vi "Upload_test_VI _20230224.vi"(8 "error in":errorcluster, 11 "SHz_selection":enum16{"10k", "100k"}(ring)) -> (0 "error out":errorcluster, 2 "selected F_array_Link":path[](array[path]), 3 "selected folder_List":string[](array[string]))   [LabVIEW 2018]
panel:
  out "present_s_path":path
  out "S_path":path[](array[path])
  in  "Server selection":u16(ring) items=["Rackstation", "QTserver", "QDserver", "D:\\", "C:\\", "SQserver"]
  in  "Add All Sample":bool
  in  "Add All":bool
  out "FOL#":i32
  out "x-1":u32
  out "SIDE":i32
  in  "Scrollbar V":i32(c297)
  out "Selected EX#":i32
  out "element":string
  in  "END":bool
  in  "All_Clear":bool
  in  "EX_IDX":i32
  out "Height":u32
  out "Top":i32
  out "Vertical":i32
  in  "selection":u16(ring) items=["backup (Rackstation)", "BR", "cadet", "COVID19", "Gynecologic Cancer", "HU", "KATO", "KATO2", "KATO3", "komoto", "Konno", "Kumamoto", "Kumamoto_N", "Lee", "Lee2", "Lee3", "LG_EX", "Lipid", "Numata_CHR", "Numata_MF", "Numata_N", "oligopeptide", "Pan_Cancer_N2", "Phi174", "Ryu", "Smoking"]
  out "1folder names":string[](array[string])
  out "Folder_List":string[](array[string])
  out "F_array_Link":path[](array[path])
  out "2folder_name":string[](array[string])
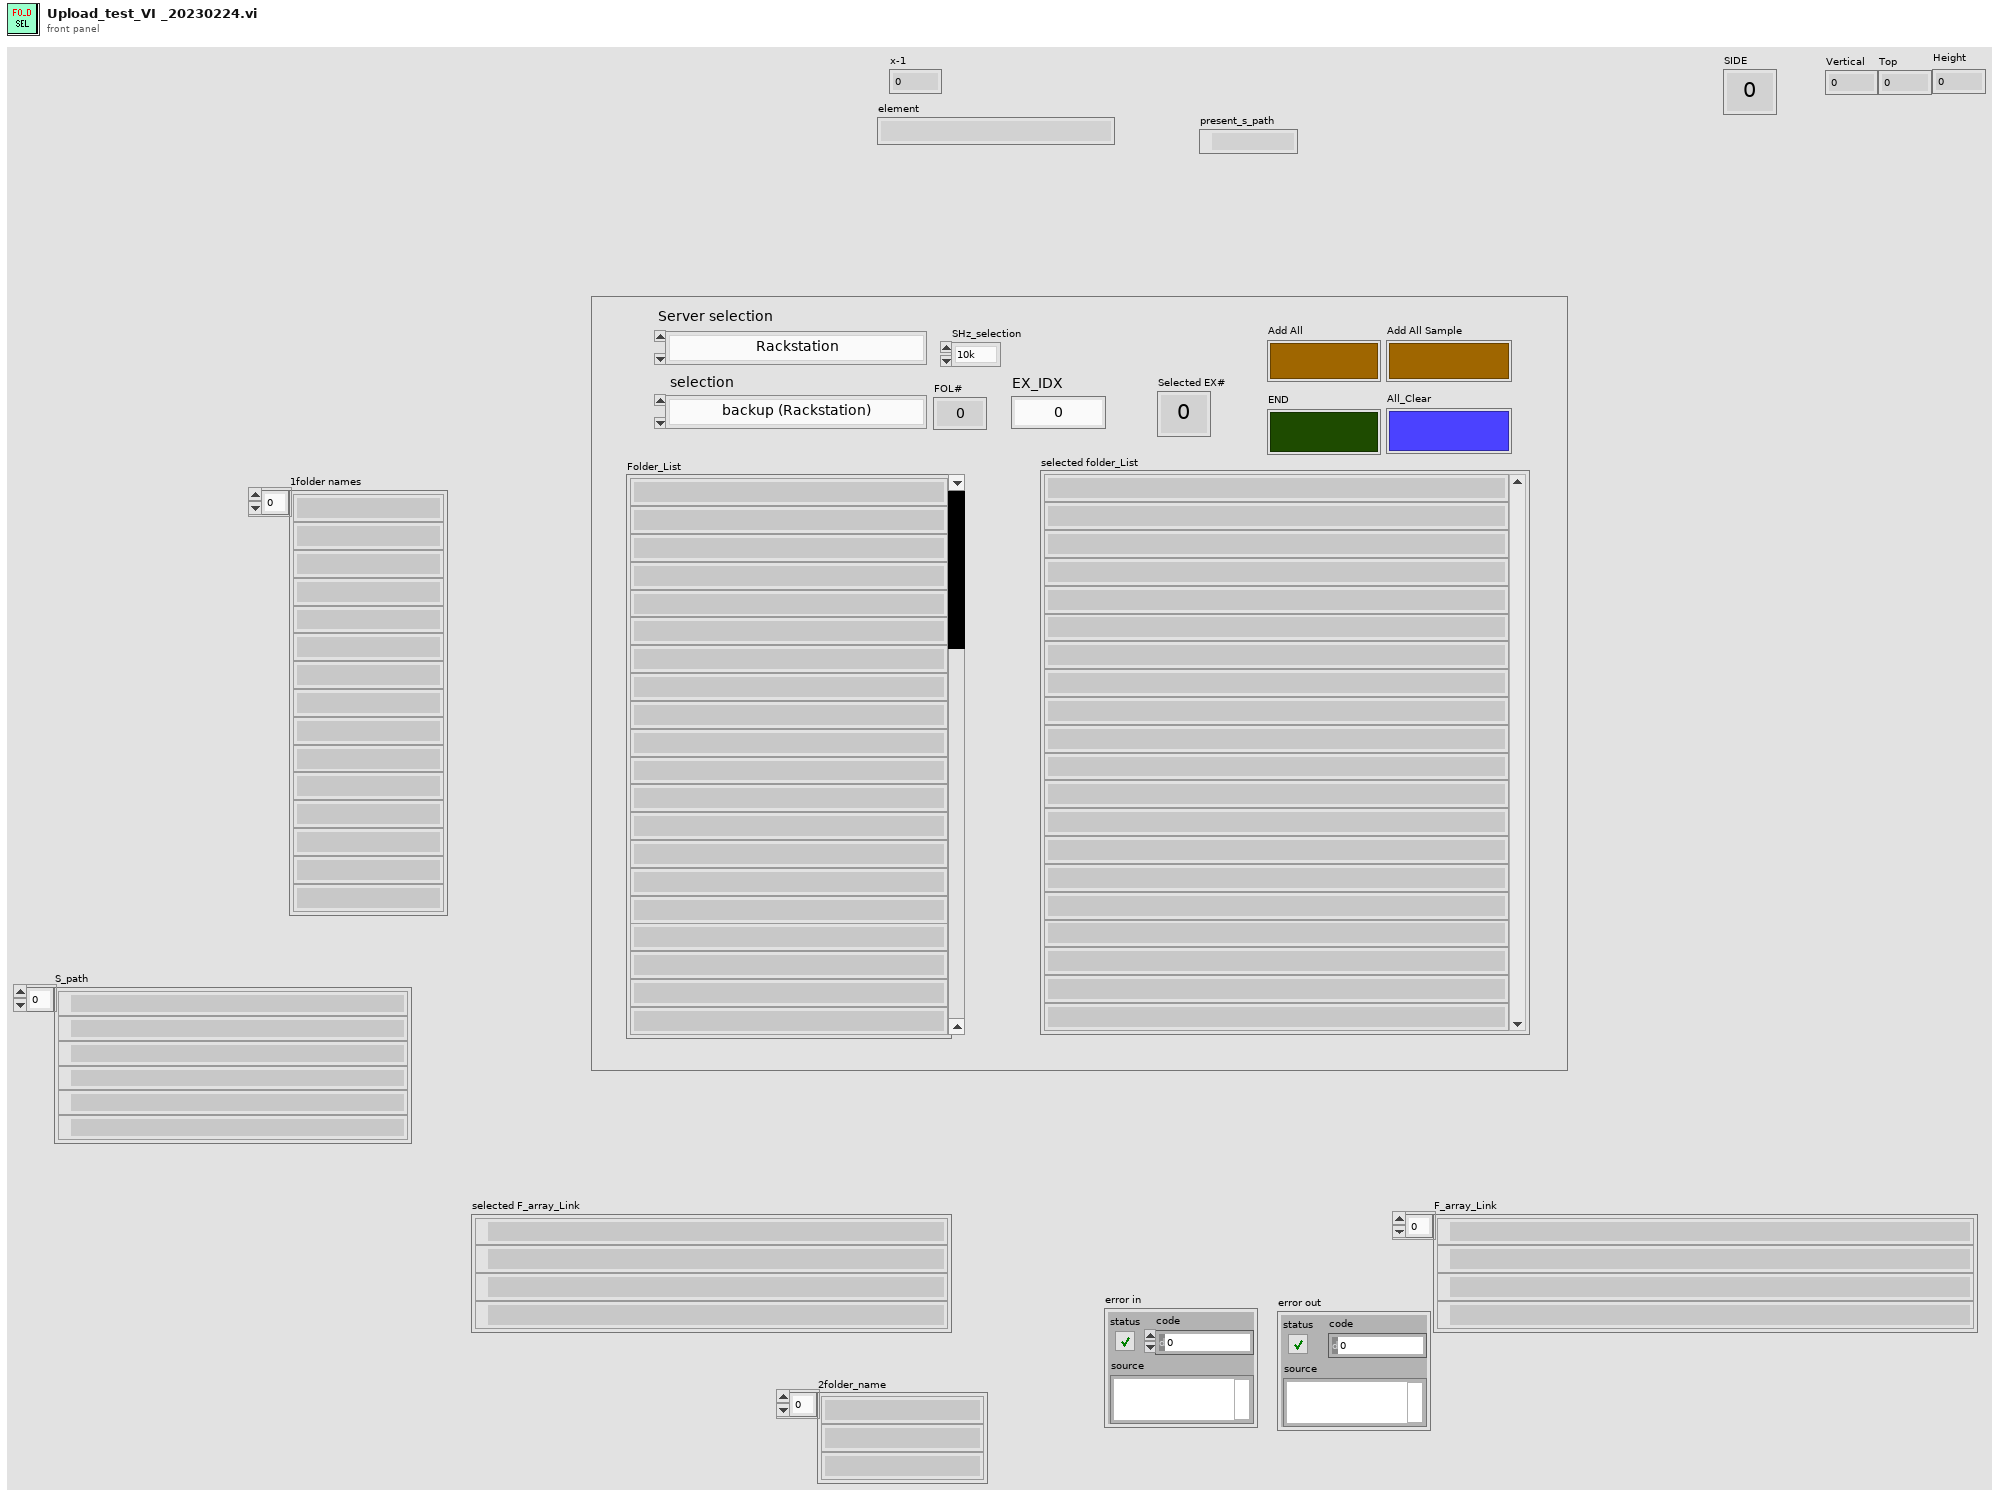
[diagram p1: front panel]
types:
  T1 = typedef "LVPoint32TypeDef.ctl" = cluster{"Horizontal":i32, "Vertical":i32}
  T2 = typedef "LVPositionTypeDef.ctl" = cluster{"Left":i32, "Top":i32}
  T3 = typedef "LVBoundsTypeDef.ctl" = cluster{"Width":u32, "Height":u32}
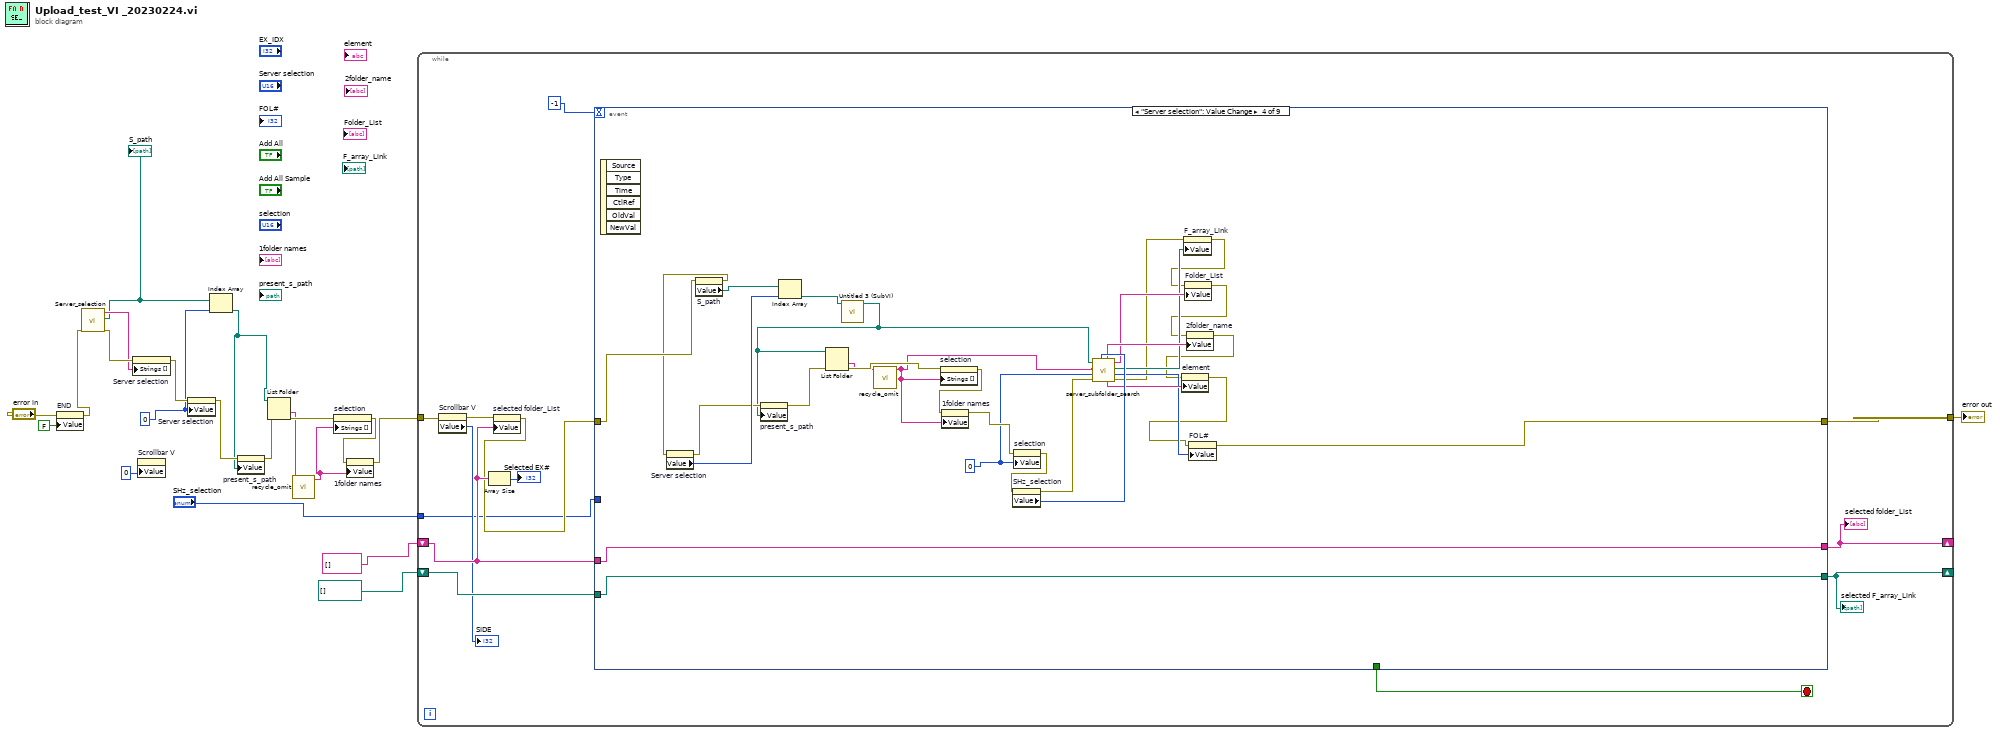
[diagram p0: block diagram]
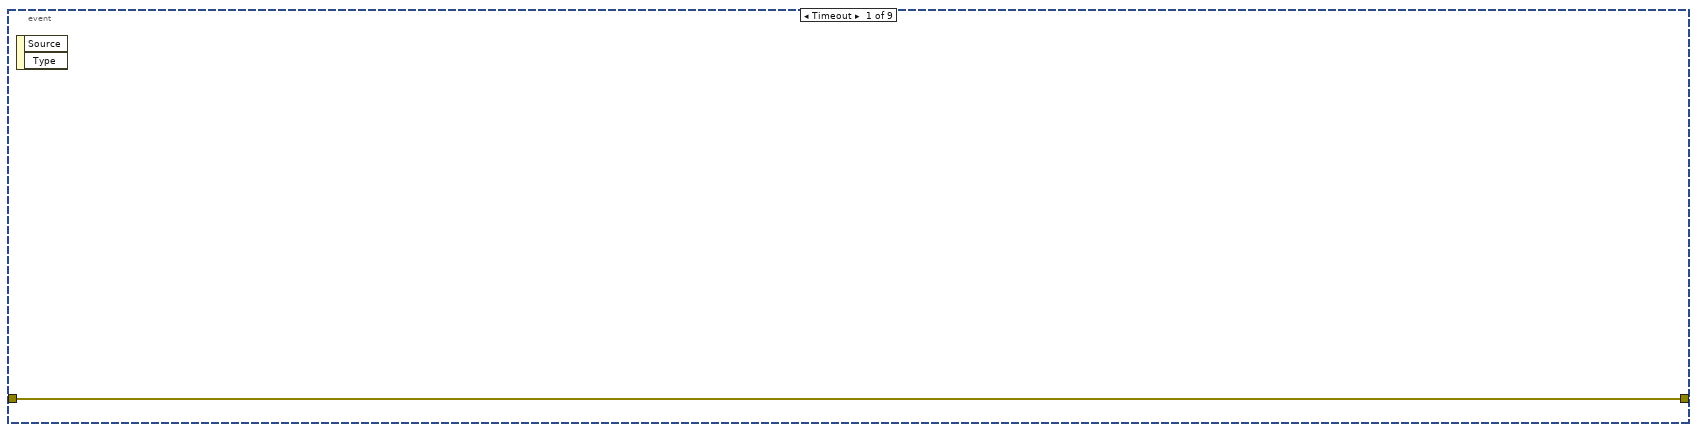
[diagram p2: hidden frame]
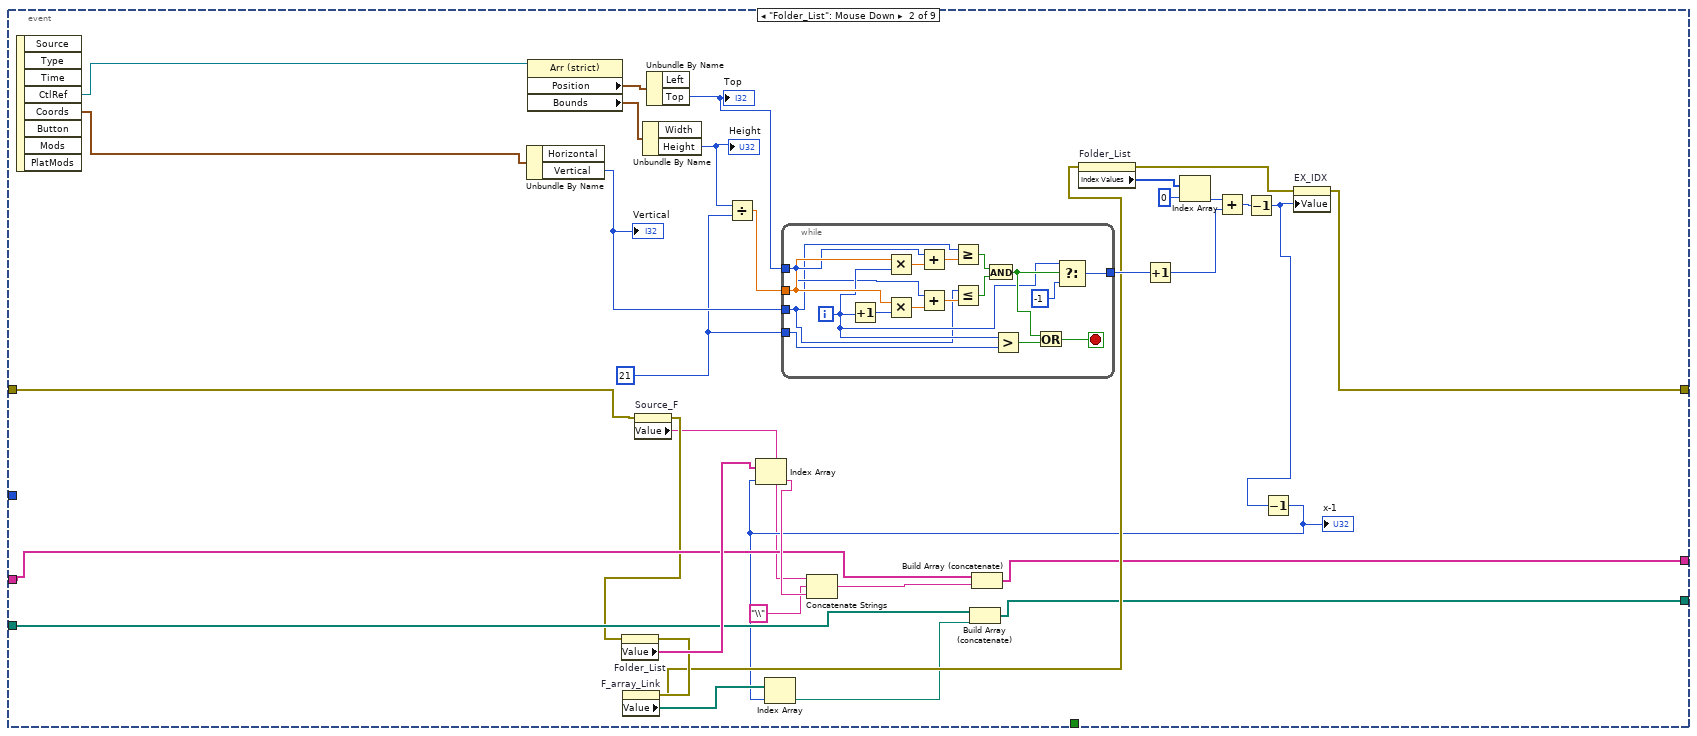
[diagram p3: hidden frame]
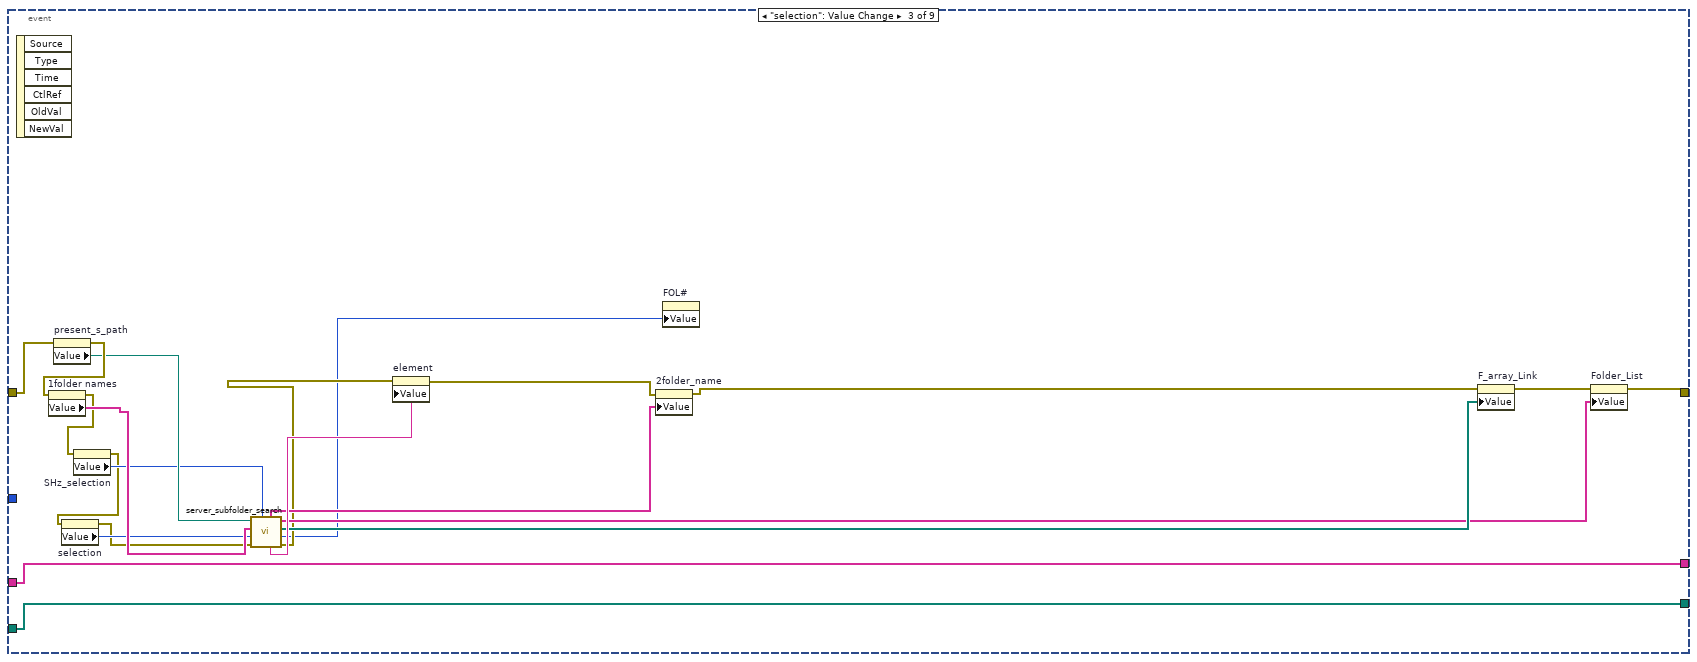
[diagram p4: hidden frame]
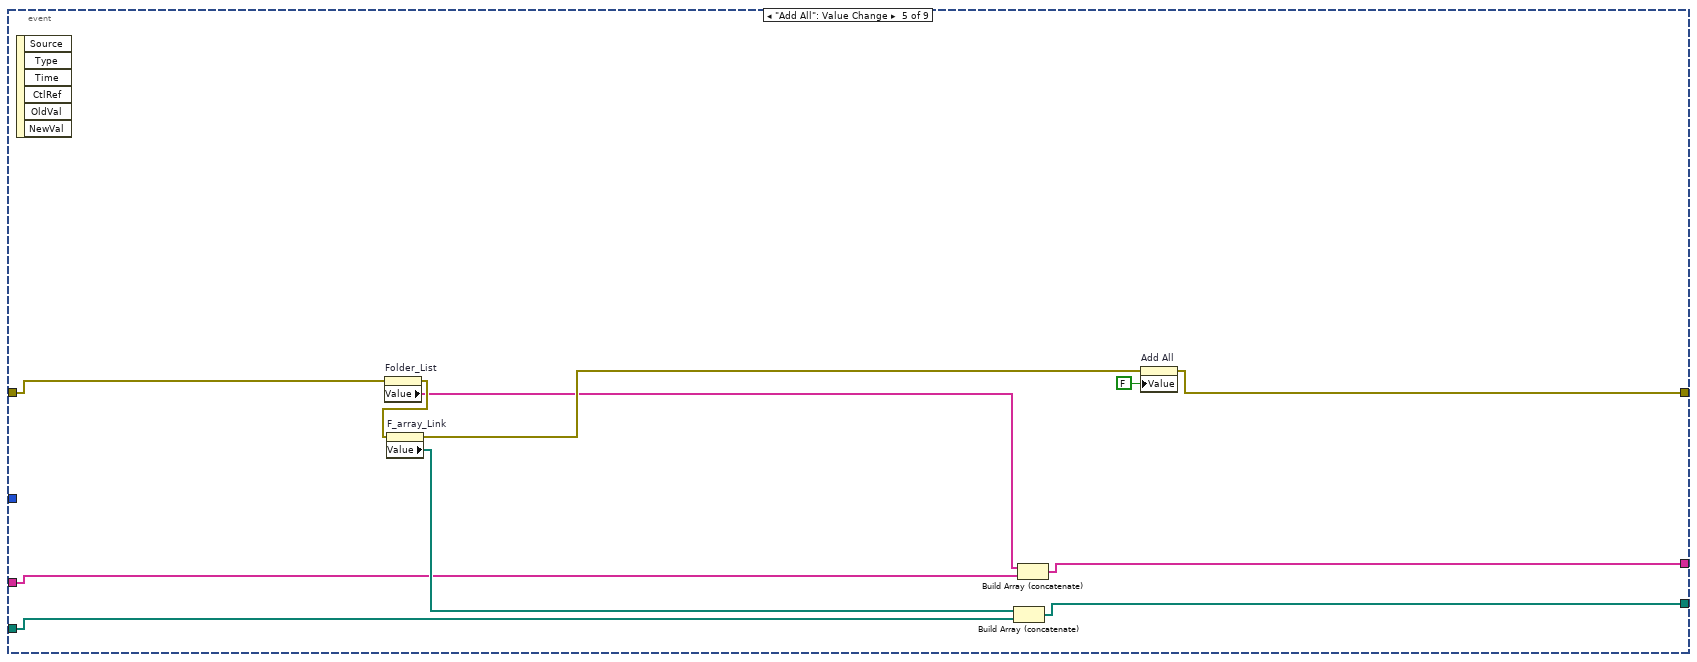
[diagram p5: hidden frame]
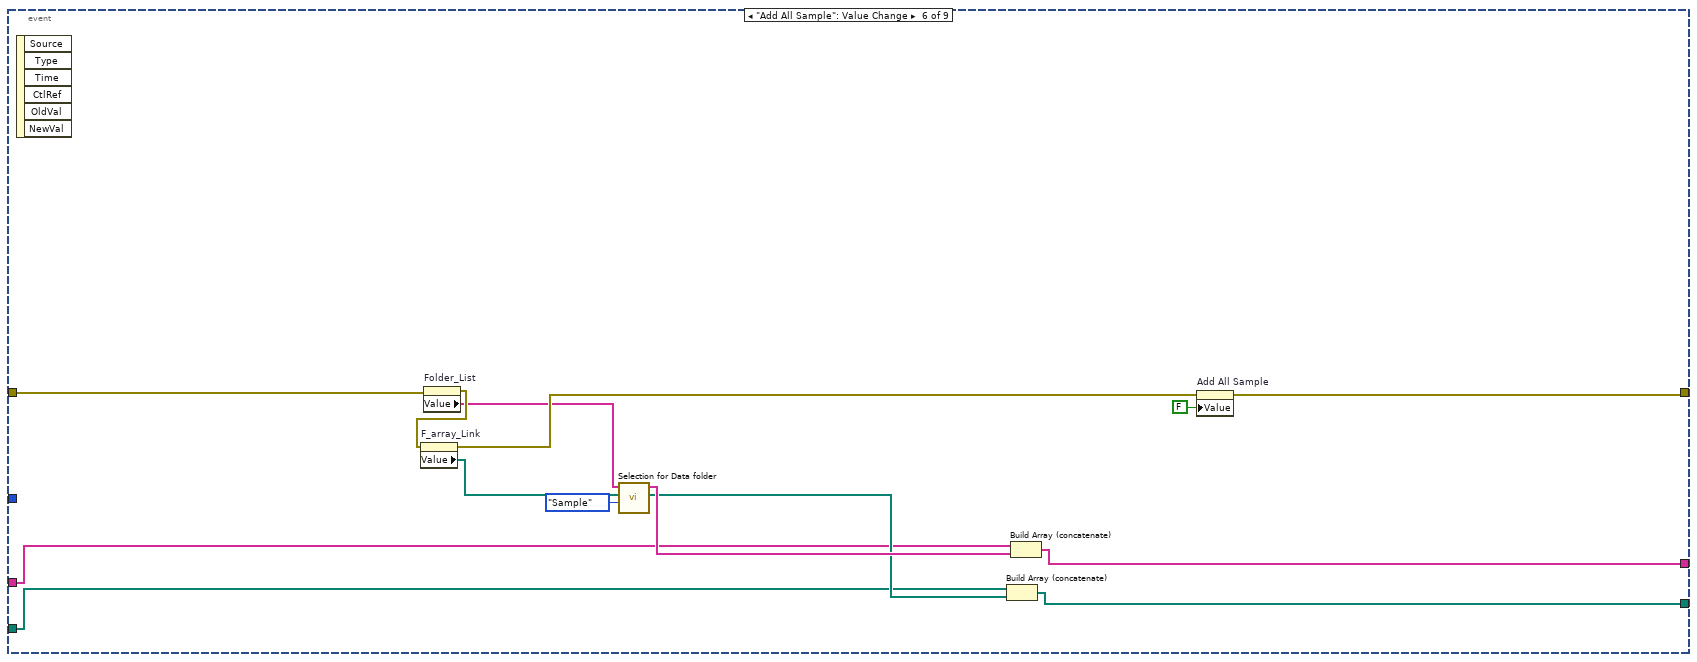
[diagram p6: hidden frame]
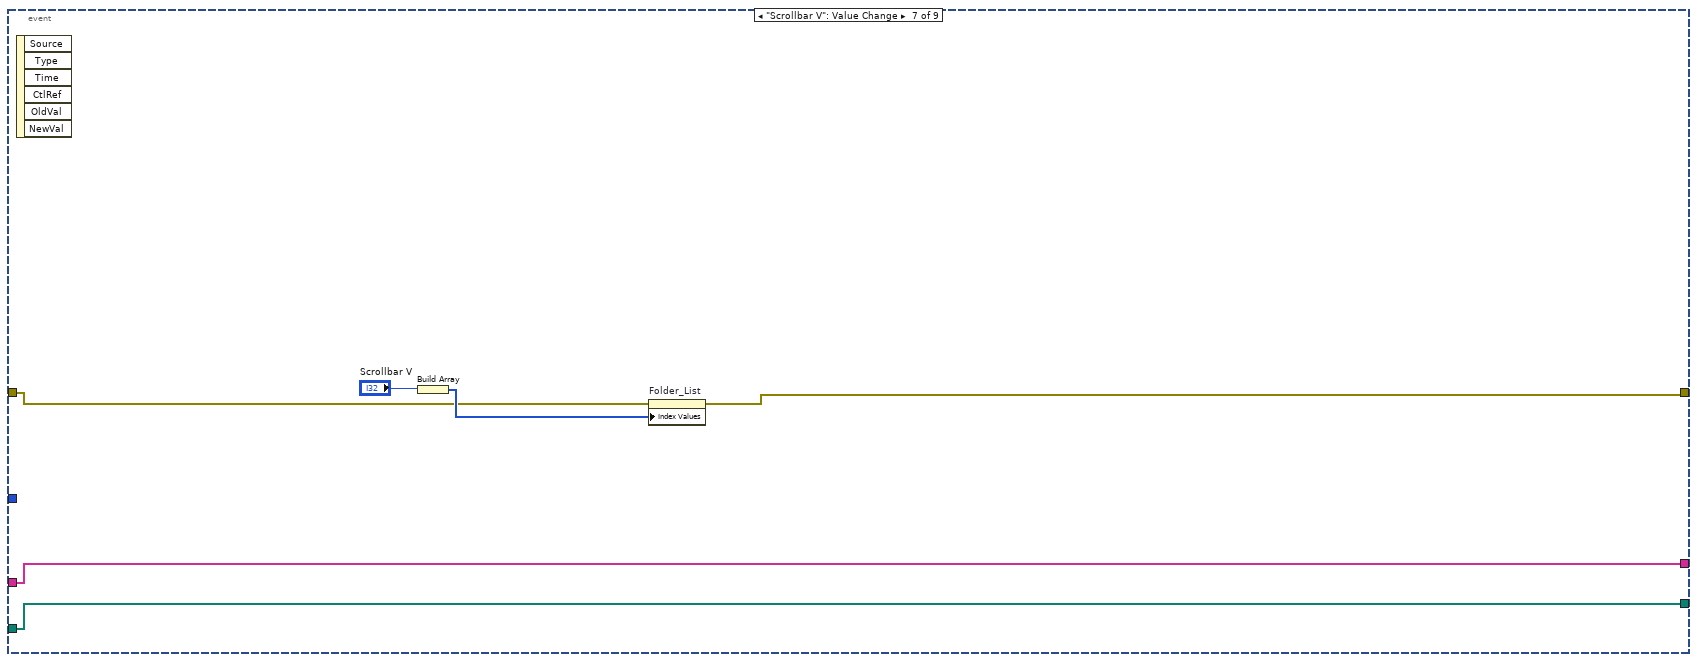
[diagram p7: hidden frame]
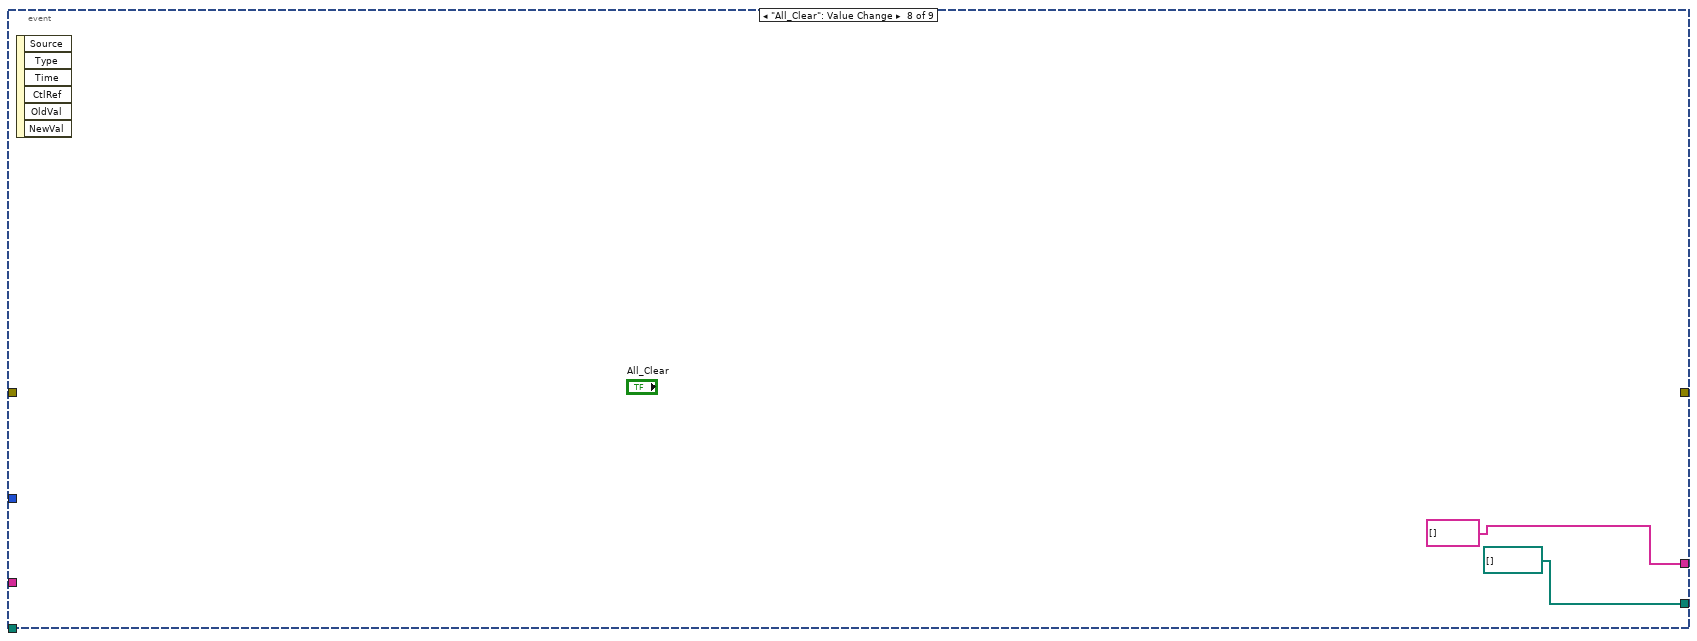
[diagram p8: hidden frame]
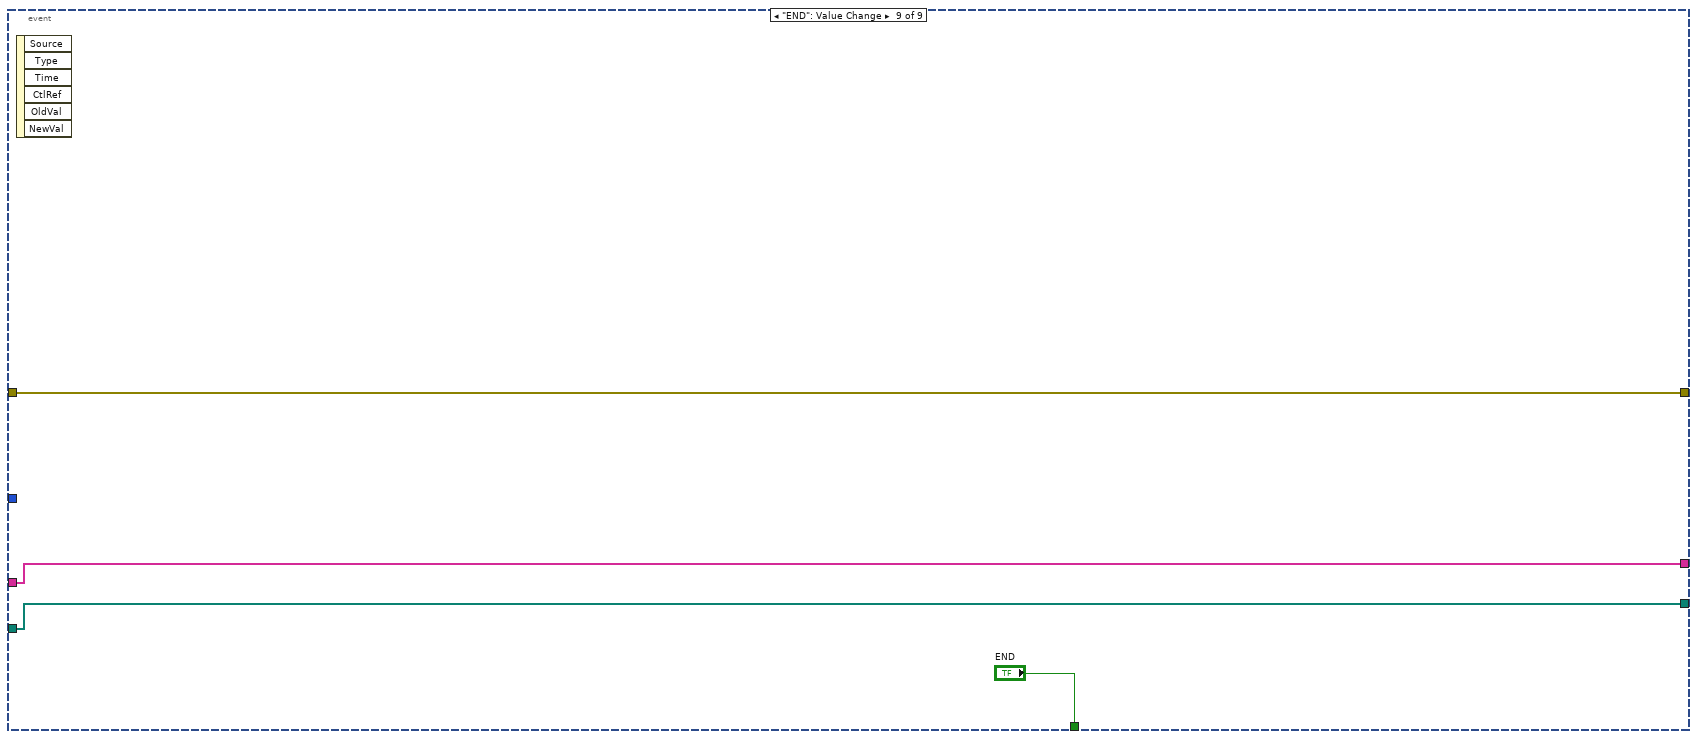
[diagram p9: hidden frame]
diagram:
  w7 = 0
  n1 = property on="END" class="Bool (strict)"(error in="error in", "Value"=FALSE ("END")) -> (error out=w12:errorcluster)  [unwired: 1 in, 1 out]
  n2 = call "Server_selection.vi"("error in (no error)"=w12) -> ("error out"=w11:errorcluster, "path 2"=w8:path[], "server_name_list"=w10:string[])  [unwired: 8 in]
  "S_path" <- w8
  n3 = property on="Server selection" class="Ring (strict)"(error in=w11, "Strings []"=w10) -> (error out=w9:errorcluster)  [unwired: 1 in, 1 out]
  n4 = property on="Scrollbar V" class="Scroll (strict)"("Value"=0 ("Scrollbar V")) -> ()  [unwired: 2 in, 2 out]
  n5 = property on="Server selection" class="Ring (strict)"(error in=w9, "Value"=w7) -> (error out=w3:errorcluster)  [unwired: 1 in, 1 out]
  n6 = Index Array(array=w8, index=w7) -> (element=w1:path)
  n7 = property on="present_s_path" class="Path"(error in=w3, "Value"=w1) -> (error out=w2:errorcluster)  [unwired: 1 in, 1 out]
  n8 = List Folder(path=w1, error in=w2) -> (folder names=w16:string[], error out=w21:errorcluster)  [unwired: 2 in, 2 out]
  n9 = call "recycle_omit.vi"("1folder names"=w16) -> ("Array"=w6:string[])  [unwired: 10 in]
  n10 = property on="selection" class="Ring (strict)"(error in=w21, "Strings []"=w6) -> (error out=w5:errorcluster)  [unwired: 1 in, 1 out]
  n11 = property on="1folder names" class="Arr (strict)"(error in=w5, "Value"=w6) -> (error out=w4:errorcluster)  [unwired: 1 in, 1 out]
  n12 = while {
    tunnel: w4 -> [w27]
    tunnel: [w34] -> w20
    shift-right: [w24] -> _
    shift-left: string[] [] -> [w29]
    shift-right: [w30] -> _
    shift-left: path[] [] -> [w31]
    tunnel: "SHz_selection" -> [w22]
    stop <- w32 stop-if-true
    n13 = property on="Scrollbar V" class="Scroll (strict)"(error in=w27) -> (error out=w26:errorcluster, "Value"=→"SIDE":i32)  [unwired: 1 in, 1 out]
    n14 = Array Size(array=w29) -> (size(s)=→"Selected EX#":i32)
    n15 = property on="selected folder_List" class="Arr (strict)"(error in=w26, "Value"=w29) -> (error out=w23:errorcluster)  [unwired: 1 in, 1 out]
    n16 = event shown="[3] \"Server selection\": Value Change" {
      selector: _ -> [_ _ _ _ _ _ _ _ _]
      dyn-events: _ -> [_ _ _ _ _ _ _ _ _]
      timeout: -1 -> [_ _ _ _ _ _ _ _ _]
      tunnel: w23 -> [w35 w39 w104 w135 w148 w161 w167 _ w171]
      tunnel: [w35 w41 w107 w108 w144 w158 w166 _ w171] -> w34
      tunnel: w29 -> [_ w44 w106 w136 w138 w149 w164 _ w173]
      tunnel: [_ w43 w106 w136 w142 w152 w164 string[] [] w173] -> w24
      tunnel: [_ _ _ _ _ _ _ _ "END"] -> w32
      tunnel: w31 -> [_ w45 w105 w137 w139 w150 w163 _ w172]
      tunnel: [_ w42 w105 w137 w141 w151 w163 path[] [] w172] -> w30
      tunnel: w22 -> [_ _ _ _ _ _ _ _ _]
      event Timeout {
        n17 = event-data() -> ()  [unwired: 1 in, 2 out]
      }
      event "Folder_List": Mouse Down {
        w49 = 21 ("f")
        n18 = event-data() -> ("CtlRef"=w46:refnum<vi>, "Coords"=w47:T1)  [unwired: 1 in, 6 out]
        n19 = Unbundle By Name(w47) -> ("Vertical"=w66:i32)  [unwired: 1 out]
        "Vertical" <- w66
        n20 = property class="Arr (strict)"(reference=w46) -> ("Position"=w68:T2, "Bounds"=w67:T3)  [unwired: 1 in, 2 out]
        n21 = property on="Source_F" class="Str"(error in=w39) -> (error out=w38:errorcluster, "Value"=w37:string)  [unwired: 1 in, 1 out]
        n22 = property on="Folder_List" class="Arr (strict)"(error in=w38) -> (error out=w54:errorcluster, "Value"=w58:string[])  [unwired: 1 in, 1 out]
        n23 = property on="F_array_Link" class="Arr (strict)"(error in=w54) -> (error out=w53:errorcluster, "Value"=w52:path[])  [unwired: 1 in, 1 out]
        n24 = Unbundle By Name(w67) -> ("Height"=w65:u32)  [unwired: 1 out]
        "Height" <- w65
        n25 = Unbundle By Name(w68) -> ("Top"=w63:i32)  [unwired: 1 out]
        "Top" <- w63
        n26 = Divide(x=w65, y=w49) -> (x/y=w64:dbl)
        n27 = while {
          tunnel: w66 -> [w70]
          tunnel: w64 -> [w76]
          tunnel: w63 -> [w72]
          tunnel: [w81] -> w59
          tunnel: w49 -> [w71]
          i -> [w75]
          stop <- w79 stop-if-true
          n28 = Increment(x=w75) -> (x+1=w86:i32)
          n29 = Multiply(x=w76, y=w75) -> (x*y=w73:dbl)
          n30 = Multiply(x=w76, y=w86) -> (x*y=w84:dbl)
          n31 = Add(x=w72, y=w73) -> (x+y=w74:dbl)
          n32 = Add(x=w72, y=w84) -> (x+y=w85:dbl)
          n33 = Greater Or Equal?(x=w70, y=w74) -> (x >= y?=w83:bool)
          n34 = Less Or Equal?(x=w70, y=w85) -> (x <= y?=w82:bool)
          n35 = And(x=w83, y=w82) -> (x .and. y?=w78:bool)
          n36 = Greater?(x=w75, y=w71) -> (0:w77:bool)
          n37 = Or(x=w78, y=w77) -> (x .or. y?=w79:bool)
          n38 = Select(t=w75, s=w78, f=-1) -> (s? t:f=w81:i32)
        }
        n39 = property on="Folder_List" class="Arr (strict)"(error in=w53) -> (error out=w56:errorcluster, "Index Values"=w69:u32[])  [unwired: 1 in, 1 out]
        n40 = Increment(x=w59) -> (x+1=w62:i32)
        n41 = Index Array(array=w69, index=0 ("指標")) -> (element=w60:u32)
        n42 = Add(x=w60, y=w62) -> (x+y=w61:u32)
        n43 = Decrement(x=w61) -> (x-1=w36:u32)
        n44 = Decrement(x=w36) -> (x-1=w40:u32)
        "x-1" <- w40
        n45 = Index Array(array=w58, index=w40) -> (element=w57:string)
        n46 = Index Array(array=w52, index=w40) -> (element=w51:path)
        n47 = Concatenate Strings(w37, "\\" ("string"), w57) -> (w55:string)
        n48 = Build Array (concatenate)(w45, w51) -> (w42:path[])
        n49 = Build Array (concatenate)(w44, w55) -> (w43:string[])
        n50 = property on="EX_IDX" class="DigNum (strict)"(error in=w56, "Value"=w36) -> (error out=w41:errorcluster)  [unwired: 1 in, 1 out]
      }
      event "selection": Value Change {
        n51 = event-data() -> ()  [unwired: 1 in, 6 out]
        n52 = property on="present_s_path" class="Path"(error in=w104) -> (error out=w103:errorcluster, "Value"=w102:path)  [unwired: 1 in, 1 out]
        n53 = property on="1folder names" class="Arr (strict)"(error in=w103) -> (error out=w88:errorcluster, "Value"=w101:string[])  [unwired: 1 in, 1 out]
        n54 = property on="SHz_selection" class="Enum (strict)"(error in=w88) -> (error out=w87:errorcluster, "Value"=w89:enum16{"10k", "100k"})  [unwired: 1 in, 1 out]
        n55 = property on="selection" class="Ring (strict)"(error in=w87) -> (error out=w99:errorcluster, "Value"=w100:u16)  [unwired: 1 in, 1 out]
        n56 = call "server_subfolder_search.vi"("SHz_selection"=w89, "error in"=w99, "selection"=w100, "1folder names"=w101, "present_s_path"=w102) -> ("error out"=w94:errorcluster, "FOL#"=w90:i32, "F_array_Link"=w96:path[], "Folder_List"=w95:string[], "element"=w98:string, "2folder_name"=w97:string[])  [unwired: 1 in]
        n57 = property on="element" class="Str"(error in=w94, "Value"=w98) -> (error out=w93:errorcluster)  [unwired: 1 in, 1 out]
        n58 = property on="2folder_name" class="Arr (strict)"(error in=w93, "Value"=w97) -> (error out=w92:errorcluster)  [unwired: 1 in, 1 out]
        n59 = property on="FOL#" class="DigNum (strict)"("Value"=w90) -> ()  [unwired: 2 in, 2 out]
        n60 = property on="F_array_Link" class="Arr (strict)"(error in=w92, "Value"=w96) -> (error out=w91:errorcluster)  [unwired: 1 in, 1 out]
        n61 = property on="Folder_List" class="Arr (strict)"(error in=w91, "Value"=w95) -> (error out=w107:errorcluster)  [unwired: 1 in, 1 out]
      }
      event "Server selection": Value Change {
        w119 = 0
        n62 = event-data() -> ()  [unwired: 1 in, 6 out]
        n63 = property on="S_path" class="Arr (strict)"(error in=w135) -> (error out=w132:errorcluster, "Value"=w134:path[])  [unwired: 1 in, 1 out]
        n64 = property on="Server selection" class="Ring (strict)"(error in=w132) -> (error out=w126:errorcluster, "Value"=w133:u16)  [unwired: 1 in, 1 out]
        n65 = Index Array(array=w134, index=w133) -> (element=w131:path)
        n66 = call "Untitled 3 (SubVI).vi"("String"=w131) -> ("Path"=w124:path)  [unwired: 10 in]
        n67 = property on="present_s_path" class="Path"(error in=w126, "Value"=w124) -> (error out=w125:errorcluster)  [unwired: 1 in, 1 out]
        n68 = List Folder(path=w124, error in=w125) -> (folder names=w129:string[], error out=w130:errorcluster)  [unwired: 2 in, 2 out]
        n69 = call "recycle_omit.vi"("1folder names"=w129) -> ("Array"=w123:string[])  [unwired: 10 in]
        n70 = property on="selection" class="Ring (strict)"(error in=w130, "Strings []"=w123) -> (error out=w128:errorcluster)  [unwired: 1 in, 1 out]
        n71 = property on="1folder names" class="Arr (strict)"(error in=w128, "Value"=w123) -> (error out=w127:errorcluster)  [unwired: 1 in, 1 out]
        n72 = property on="selection" class="Ring (strict)"(error in=w127, "Value"=w119) -> (error out=w122:errorcluster)  [unwired: 1 in, 1 out]
        n73 = property on="SHz_selection" class="Enum (strict)"(error in=w122) -> (error out=w121:errorcluster, "Value"=w120:enum16{"10k", "100k"})  [unwired: 1 in, 1 out]
        n74 = call "server_subfolder_search.vi"("SHz_selection"=w120, "error in"=w121, "selection"=w119, "1folder names"=w123, "present_s_path"=w124) -> ("error out"=w113:errorcluster, "FOL#"=w114:i32, "F_array_Link"=w115:path[], "Folder_List"=w116:string[], "element"=w117:string, "2folder_name"=w118:string[])  [unwired: 1 in]
        n75 = property on="F_array_Link" class="Arr (strict)"(error in=w113, "Value"=w115) -> (error out=w112:errorcluster)  [unwired: 1 in, 1 out]
        n76 = property on="Folder_List" class="Arr (strict)"(error in=w112, "Value"=w116) -> (error out=w111:errorcluster)  [unwired: 1 in, 1 out]
        n77 = property on="2folder_name" class="Arr (strict)"(error in=w111, "Value"=w118) -> (error out=w110:errorcluster)  [unwired: 1 in, 1 out]
        n78 = property on="element" class="Str"(error in=w110, "Value"=w117) -> (error out=w109:errorcluster)  [unwired: 1 in, 1 out]
        n79 = property on="FOL#" class="DigNum (strict)"(error in=w109, "Value"=w114) -> (error out=w108:errorcluster)  [unwired: 1 in, 1 out]
      }
      event "Add All": Value Change {
        n80 = event-data() -> ()  [unwired: 1 in, 6 out]
        n81 = property on="Folder_List" class="Arr (strict)"(error in=w148) -> (error out=w147:errorcluster, "Value"=w143:string[])  [unwired: 1 in, 1 out]
        n82 = property on="F_array_Link" class="Arr (strict)"(error in=w147) -> (error out=w146:errorcluster, "Value"=w140:path[])  [unwired: 1 in, 1 out]
        n83 = Build Array (concatenate)(w140, w139) -> (w141:path[])
        n84 = Build Array (concatenate)(w143, w138) -> (w142:string[])
        n85 = property on="Add All" class="Bool (strict)"(error in=w146, "Value"=FALSE ("Add All")) -> (error out=w144:errorcluster)  [unwired: 1 in, 1 out]
      }
      event "Add All Sample": Value Change {
        n86 = event-data() -> ()  [unwired: 1 in, 6 out]
        n87 = property on="Folder_List" class="Arr (strict)"(error in=w161) -> (error out=w160:errorcluster, "Value"=w157:string[])  [unwired: 1 in, 1 out]
        n88 = property on="F_array_Link" class="Arr (strict)"(error in=w160) -> (error out=w159:errorcluster, "Value"=w156:path[])  [unwired: 1 in, 1 out]
        n89 = call "Selection for Data folder.vi"("Select"=enum16{"Sample", "Blank"}."Sample", "F_array_Link"=w156, "Folder_List"=w157) -> ("S_F_array_Link"=w153:path[], "S_Folder_List"=w154:string[])  [unwired: 7 in]
        n90 = Build Array (concatenate)(w150, w153) -> (w151:path[])
        n91 = Build Array (concatenate)(w149, w154) -> (w152:string[])
        n92 = property on="Add All Sample" class="Bool (strict)"(error in=w159, "Value"=FALSE ("Add All Sample")) -> (error out=w158:errorcluster)  [unwired: 1 in, 1 out]
      }
      event "Scrollbar V": Value Change {
        n93 = event-data() -> ()  [unwired: 1 in, 6 out]
        n94 = Build Array("Scrollbar V") -> (w168:i32[])
        n95 = property on="Folder_List" class="Arr (strict)"(error in=w167, "Index Values"=w168) -> (error out=w166:errorcluster)  [unwired: 1 in, 1 out]
      }
      event "All_Clear": Value Change {
        n96 = event-data() -> ()  [unwired: 1 in, 6 out]
      }
      event "END": Value Change {
        n97 = event-data() -> ()  [unwired: 1 in, 6 out]
      }
    }
    "selected F_array_Link" <- w30
    "selected folder_List" <- w24
  }
  "error out" <- w20
